vi "Add Line.vi"(8 "error in":errorcluster, 10 "Line":T1, 11 "UI Reference configuration in":refnum<class "UI Reference configuration.lvclass">) -> (0 "error out":errorcluster, 2 "Line Index":i32, 3 "UI Reference configuration out":refnum<class "UI Reference configuration.lvclass">)   [LabVIEW 2015, in "UI Reference configuration.lvclass"]
doc: "Adds a new line to a configuration."
uses:
  UI Reference configuration.lvclass
  Line.ctl
  <vilib>/NI/Tag Bus Module Framework/channel/TBM channel.lvclass
  UI Reference configuration.lvclass/UI Reference configuration.ctl
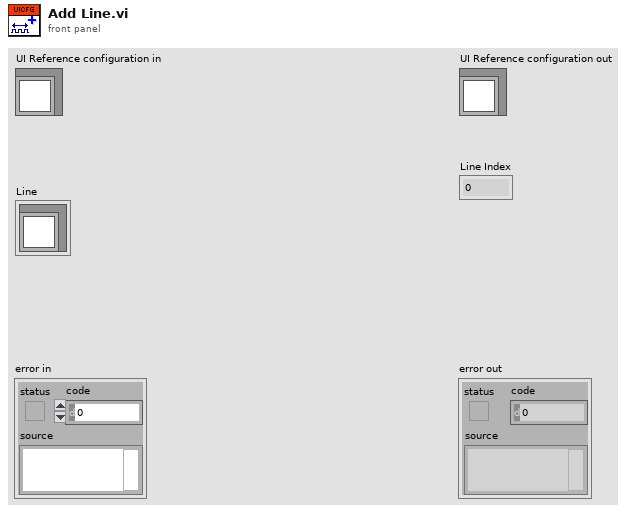
[diagram p1: front panel]
types:
  T1 = typedef "UI Reference configuration.lvclass/Line.ctl" = cluster{"channel":refnum<class "TBM channel.lvclass">}
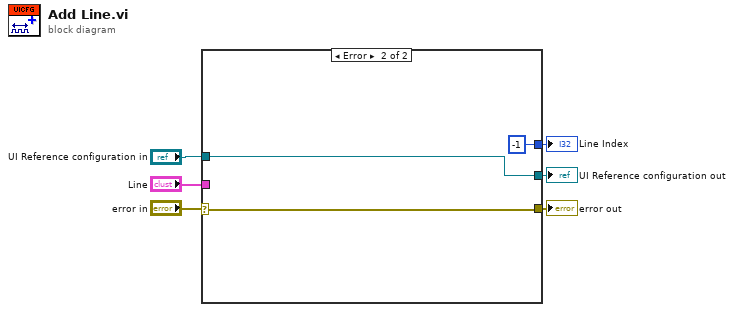
[diagram p0: block diagram]
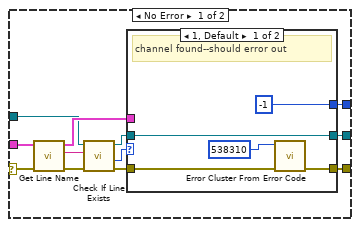
[diagram p2: hidden frame]
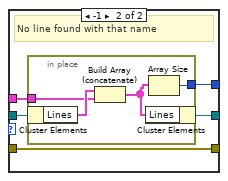
[diagram p3: hidden frame]
diagram:
  n1 = case shown="Error" "error in" {
    selector: "error in" -> [w8 w33]
    tunnel: [w18 w33] -> w6
    tunnel: [w17 w34] -> w5
    tunnel: "Line" -> [w13 _]
    tunnel: [w9 -1] -> w3
    tunnel: "UI Reference configuration in" -> [w7 w34]
    frame No Error {
      n2 = call "Get Line Name.vi"("error in"=w8, "Line in"=w13) -> ("error out"=w15:errorcluster, "Name"=w14:string, "Line out"=w12:T1)  [unwired: 7 in]
      n3 = call-dynamic "Check If Line Exists.vi"("error in"=w15, "Name to Locate"=w14, "UI Reference configuration in"=w7) -> ("error out"=w16:errorcluster, "Index"=w11:i32, "UI Reference configuration out"=w10:refnum<class "UI Reference configuration.lvclass">)  [unwired: 4 in, 2 out]
      n4 = case shown="1, Default" w11 {
        tunnel: [w23 w27] -> w18
        tunnel: w16 -> [w21 w27]
        tunnel: w10 -> [w20 w26]
        tunnel: w12 -> [_ w28]
        tunnel: [w20 w25] -> w17
        tunnel: [-1 w24] -> w9
        frame 1, Default {
          # "channel found--should error out"
          n5 = call <vilib>:"Error Cluster From Error Code.vi"("error in (no error)"=w21, "error code (0)"=538310) -> ("error out"=w23:errorcluster)  [unwired: 7 in]
        }
        frame -1 {
          # "No line found with that name"
          n6 = in-place {
            in-place-border: w28 -> [w31]
            in-place-border: [w29] -> w24
            n7 = in-place-cluster #1(w26) -> ("Lines"=w32:T1[])
            n8 = Build Array (concatenate)(w32, w31) -> (w30:T1[])
            n9 = in-place-cluster #1("Lines"=w30) -> (w25:refnum<class "UI Reference configuration.lvclass">)
            n10 = Array Size(array=w30) -> (size(s)=w29:i32)
          }
        }
      }
    }
    frame Error {
    }
  }
  "error out" <- w6
  "UI Reference configuration out" <- w5
  "Line Index" <- w3
